vi "initialize.vi"(8 "error in (no error)":errorcluster, 11 "Mechanism in":refnum<class "Mechanism.lvclass">) -> (0 "error out":errorcluster, 3 "Mechanism out":refnum<class "Mechanism.lvclass">)   [LabVIEW 2018, in "Mechanism.lvclass"]
uses:
  Mechanism.lvclass
  Mechanism.lvclass/Mechanism.ctl
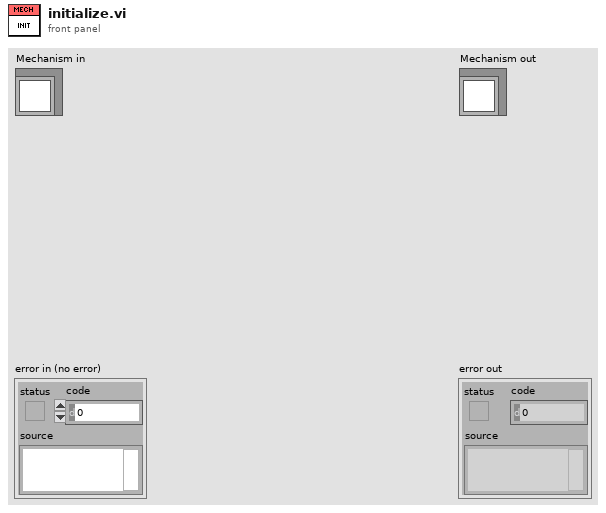
[diagram p1: front panel]
types:
  T1 = cluster{"mode":string, "condition":string, "position":string, "pos_name":string, "pos_id":string}
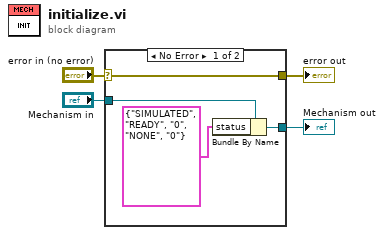
[diagram p0: block diagram]
diagram:
  n1 = case shown="No Error" "error in (no error)" {
    selector: "error in (no error)" -> [w8 w10]
    tunnel: [w8 w10] -> w3
    tunnel: [w6 w9] -> w1
    tunnel: "Mechanism in" -> [w7 w9]
    frame No Error {
      n2 = Bundle By Name(cluster=w7, "status"=T1 {"mode"="SIMULATED", "condition"="READY", "position"="0", "pos_name"="NONE", "pos_id"="0"}) -> (w6:refnum<class "Mechanism.lvclass">)
    }
    frame Error {
    }
  }
  "error out" <- w3
  "Mechanism out" <- w1
